vi "BNAL Tdms opne intial_MS.vi"(8 "error in":errorcluster caption="エラー入力（エラーなし）", 10 "Tag cluster_B":T1, 11 "TDMSファイル入力":refnum<k34>) -> (0 "error out":errorcluster caption="エラー出力", 3 "A TDMSファイル出力":refnum<k34>)   [LabVIEW 2018]
panel:
  out "LAP Table Tag":string[](array[string])
  out "BS Table Tag":string[](array[string])
  out "LTP Table Tag":string[](array[string])
  out "LSP Table Tag":string[](array[string])
  out "LCP Table Tag":string[](array[string])
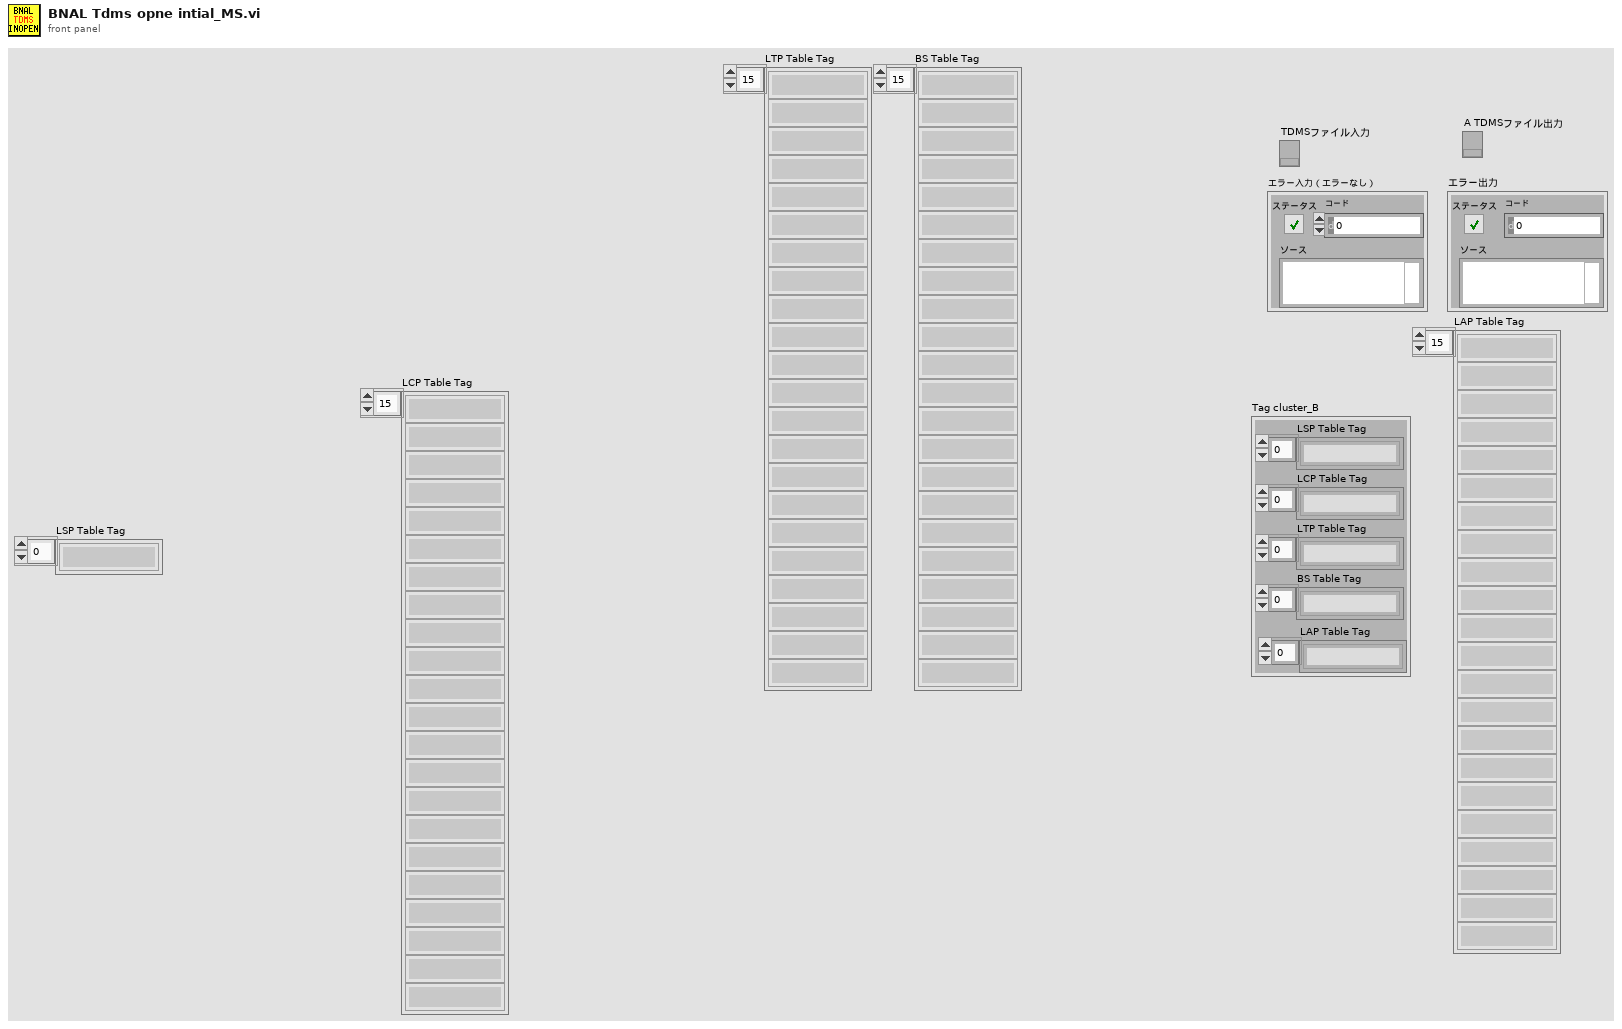
[diagram p1: front panel]
types:
  T1 = cluster{"LSP Table Tag":string[], "LCP Table Tag":string[], "LTP Table Tag":string[], "BS Table Tag":string[], "LAP Table Tag":string[]}
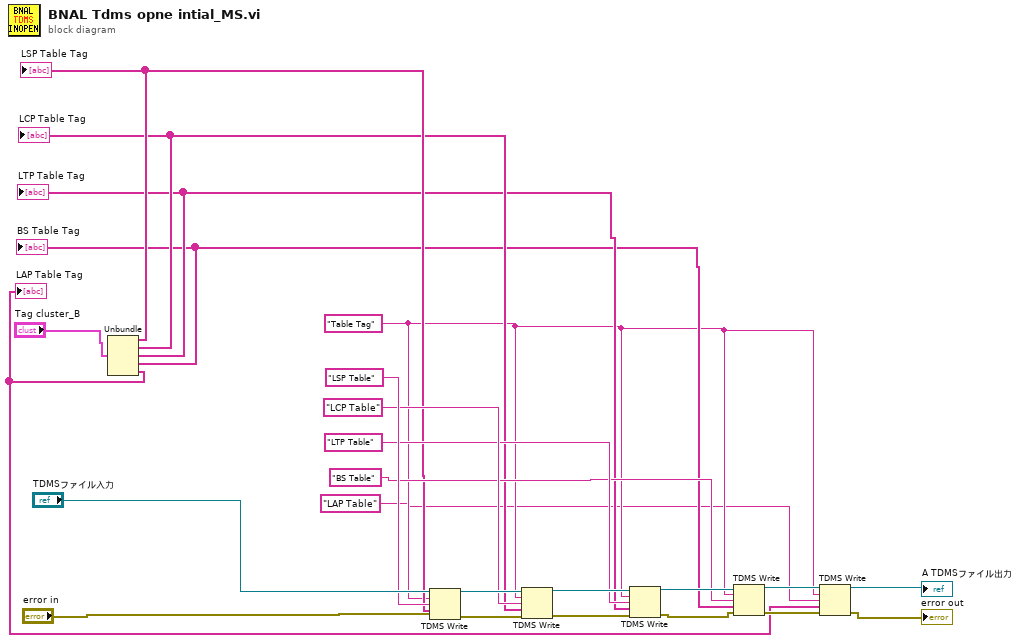
[diagram p0: block diagram]
diagram:
  w3 = "Table Tag" ("グループ名入力（名称未設定）")
  n1 = Unbundle("Tag cluster_B") -> ("LSP Table Tag"=w7:string[], "LCP Table Tag"=w6:string[], "LTP Table Tag"=w5:string[], "BS Table Tag"=w4:string[], "LAP Table Tag"=w1:string[])
  "LCP Table Tag" <- w6
  "LSP Table Tag" <- w7
  "LTP Table Tag" <- w5
  "BS Table Tag" <- w4
  "LAP Table Tag" <- w1
  n2 = TDMS Write(0:"TDMSファイル入力", 5:w3, 7:"LSP Table" ("チャンネル名入力（名称未設定）"), 9:w7, 11:"error in") -> (4:w23:refnum<k34>, 15:w24:errorcluster)  [unwired: 1 in, 2 out]
  n3 = TDMS Write(0:w23, 5:w3, 7:"LCP Table" ("チャンネル名入力（名称未設定）"), 9:w6, 11:w24) -> (4:w17:refnum<k34>, 15:w18:errorcluster)  [unwired: 1 in, 2 out]
  n4 = TDMS Write(0:w17, 5:w3, 7:"LTP Table" ("チャンネル名入力（名称未設定）"), 9:w5, 11:w18) -> (4:w16:refnum<k34>, 15:w13:errorcluster)  [unwired: 1 in, 2 out]
  n5 = TDMS Write(0:w16, 5:w3, 7:"BS Table" ("チャンネル名入力（名称未設定）"), 9:w4, 11:w13) -> (4:w11:refnum<k34>, 15:w9:errorcluster)  [unwired: 1 in, 2 out]
  n6 = TDMS Write(0:w11, 5:w3, 7:"LAP Table" ("チャンネル名入力（名称未設定）"), 9:w1, 11:w9) -> (4:→"A TDMSファイル出力":refnum<k34>, 15:→"error out":errorcluster)  [unwired: 1 in, 2 out]
